vi "build-app.vi"(0 "project path":string, 5 "build spec":string) -> (4 "outputs":string, 6 "error code":i32, 8 "error message":string, 10 "Done":bool)   [LabVIEW 2026]
doc: "Runs one build specification of a LabVIEW project through NI's BuildTargetBuildSpecification.vi on target My Computer. Takes the project path and the build spec name as strings and reports outputs (generated files joined by LF), error code and error message as plain values for a VI Server client. An empty build spec returns error code 1 and 'no build spec given' without building. On an error, error message is the error source up to its first blank line. Done is written FALSE first and TRUE last."
uses:
  <vilib>/Utility/error.llb/Trim Whitespace One-Sided.vi
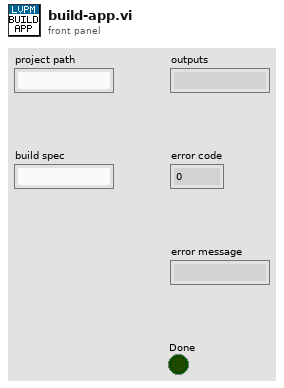
[diagram p1: front panel]
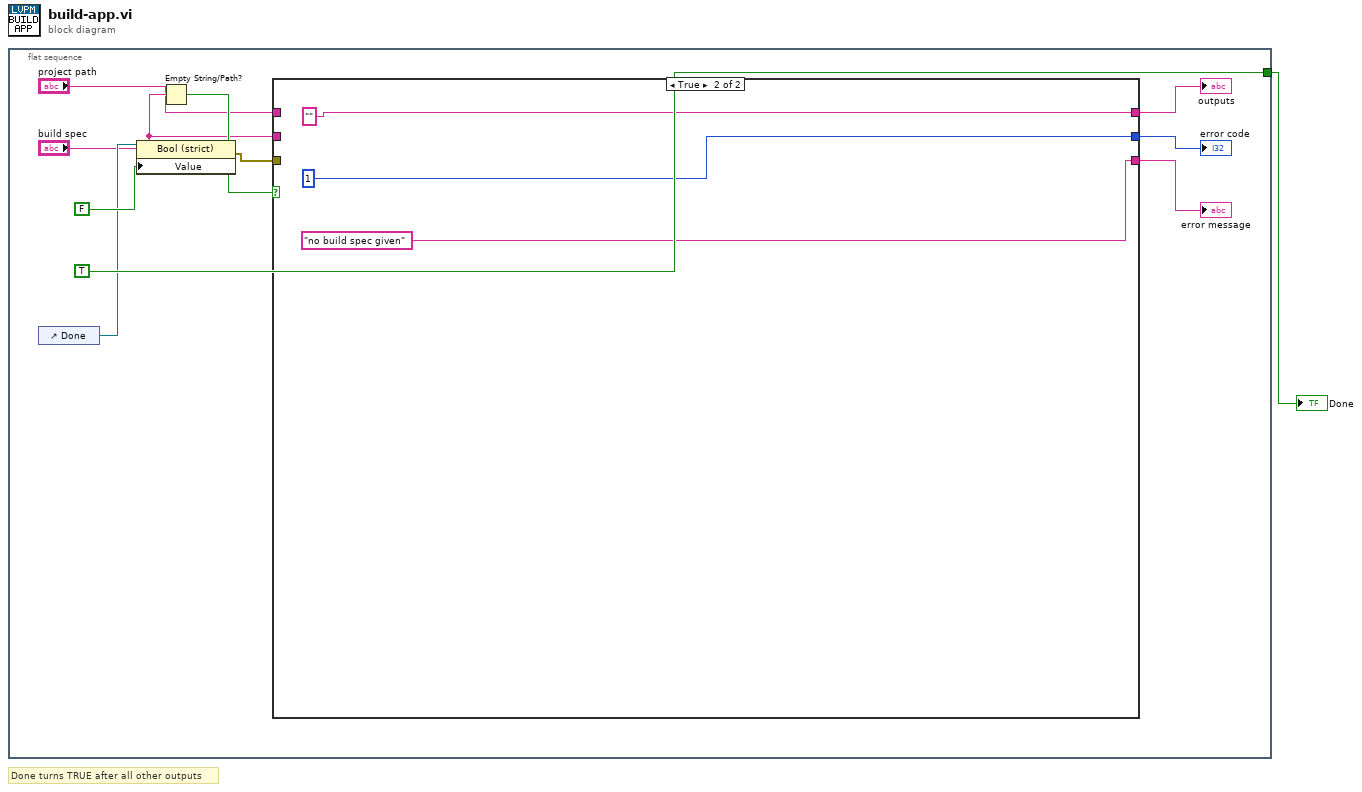
[diagram p0: block diagram]
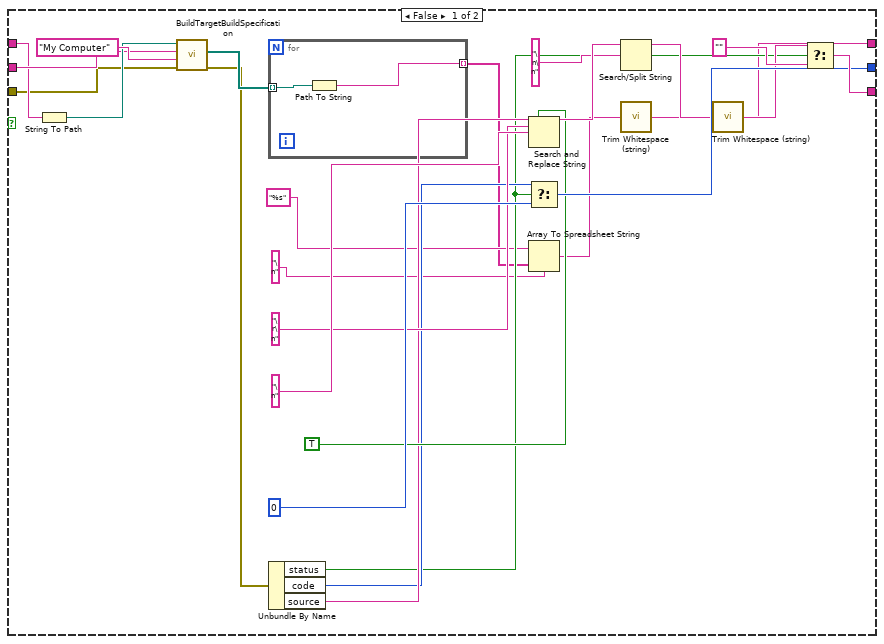
[diagram p2: hidden frame]
diagram:
  # "Done turns TRUE after all other outputs"
  n1 = flat-sequence {
    tunnel: [TRUE] -> w1
    frame #0 {
      n2 = control-ref of="Done"() -> (w4:refnum<vi>)
      n3 = property class="Bool (strict)"(reference=w4, "Value"=FALSE) -> (error out=w6:errorcluster)  [unwired: 1 in, 1 out]
      n4 = Empty String/Path?(string/path="build spec") -> (empty?=w7:bool)
      n5 = case shown="True" w7 {
        tunnel: "project path" -> [w13 _]
        tunnel: "build spec" -> [w14 _]
        tunnel: [w23 ""] -> w8
        tunnel: [w36 1] -> w9
        tunnel: [w37 "no build spec given"] -> w10
        tunnel: w6 -> [w12 _]
        frame False {
          n6 = String To Path(string=w13) -> (path=w15:path)
          n7 = call <vilib>:"BuildTargetBuildSpecification.vi"("error in (no error)"=w12, "Name of target (My Computer)"="My Computer", "Name of build specification (if empty: build all)"=w14, "Path to project"=w15) -> ("error out"=w17:errorcluster, "Generated files"=w18:path[])  [unwired: 6 in]
          n8 = for {
            tunnel: w18 -> [w38] mode=indexing
            tunnel: [w39] -> w19 mode=indexing
            n9 = Path To String(path=w38) -> (string=w39:string)
          }
          n10 = Unbundle By Name(w17) -> ("status"=w24:bool, "code"=w25:i32, "source"=w26:string)
          n11 = Search and Replace String(replace all?=TRUE, input string=w26, search string="\r\n", replace string="\n") -> (result string=w31:string)  [unwired: 4 in, 3 out]
          n12 = Select(t=w25, s=w24, f=0) -> (s? t:f=w36:i32)
          n13 = Array To Spreadsheet String(delimiter (Tab)="\n", array=w19, 3:"%s") -> (spreadsheet string=w22:string)
          n14 = Search/Split String(string=w31, search string/char (-)="\n\n") -> (substring before match=w32:string)  [unwired: 1 in, 2 out]
          n15 = call <vilib>:"Trim Whitespace (string).vi"("string"=w22) -> ("trimmed string"=w23:string)  [unwired: 1 in]
          n16 = call <vilib>:"Trim Whitespace (string).vi"("string"=w32) -> ("trimmed string"=w33:string)  [unwired: 1 in]
          n17 = Select(t=w33, s=w24, f="") -> (s? t:f=w37:string)
        }
        frame True {
        }
      }
      "outputs" <- w8
      "error code" <- w9
      "error message" <- w10
    }
  }
  "Done" <- w1
